vi "Main_RT_V2.vi"() -> ()   [LabVIEW 2018]
uses:
  enum_Main_RT_V2.ctl
  <vilib>/Platform/TimedLoop/XDataNode/timing_clust.ctl
  <vilib>/Platform/TimedLoop/XDataNode/nitl_modes.ctl
  <vilib>/Platform/TimedLoop/XDataNode/wakeup.ctl
  enum_bras.ctl
  <vilib>/myRIO/Instrument Drivers/Onboard IO/DIO/typedefs/DIO Reference.ctl
  <vilib>/myRIO/Common/Instrument Driver Framework/Utilities/typedefs/myRIO Generic Hardware Reference.ctl
  <vilib>/myRIO/Common/Instrument Driver Framework/Utilities/typedefs/Hardware Version Enum.ctl
  <vilib>/myRIO/Common/Instrument Driver Framework/Utilities/typedefs/myRIO v1.0 Reference.ctl
  <vilib>/myRIO/Common/Instrument Driver Framework/Utilities/typedefs/Generic FPGA Reference.ctl
  <vilib>/myRIO/Common/Instrument Driver Framework/myRIO v1.0/DIO/typedefs/DIO Channels List.ctl
  <vilib>/myRIO/Common/Instrument Driver Framework/myRIO v1.0/DIO/typedefs/DIO Channels Enum.ctl
  <vilib>/userdefined/High Color/nirio_resource_hc.ctl
  enum_RT_Virage.ctl
  enum_RT_Seaux.ctl
  enum_RT_recule.ctl
  enum_RT_trieur_Balles.ctl
  enum_RT_lanceur.ctl
  <vilib>/myRIO/Common/Instrument Driver Framework/Utilities/vis/Is FPGA Ref Available.vi
  <vilib>/myRIO/Common/Instrument Driver Framework/myRIO v1.0/DIO/vis/myRIO v1.1 Open DIO.vi
  <vilib>/myRIO/Instrument Drivers/Onboard IO/DIO/vis/Read.vi
  <vilib>/myRIO/Instrument Drivers/Onboard IO/DIO/vis/Write.vi
  <vilib>/myRIO/Common/Instrument Driver Framework/Utilities/vis/Validate Channels.vi
  <vilib>/myRIO/Common/Instrument Driver Framework/myRIO v1.0/DIO/vis/myRIO v1.0 Reserve DIO.vi
  <vilib>/myRIO/Common/Instrument Driver Framework/myRIO v1.0/Resource Manager/vis/myRIO v1.0 Reserve Channel List.vi
  <vilib>/myRIO/Common/Instrument Driver Framework/myRIO v1.0/DIO/vis/myRIO v1.0 Build MUX Configuration DIO.vi
  <vilib>/myRIO/Common/Instrument Driver Framework/myRIO v1.0/Resource Manager/vis/myRIO v1.0 Reserve Channel.vi
  <vilib>/myRIO/Common/Instrument Driver Framework/myRIO v1.0/Resource Manager/vis/myRIO v1.0 Unreserve Channel.vi
  <vilib>/myRIO/Common/Instrument Driver Framework/myRIO v1.0/Resource Manager/vis/myRIO v1.0 Create Configuration List.vi
  <vilib>/myRIO/Common/Instrument Driver Framework/myRIO v1.0/Resource Manager/vis/myRIO v1.0 Build Mutex Name.vi
  <vilib>/Utility/VariantDataType/GetNumericInfo.vi
  <vilib>/Utility/error.llb/Error Cluster From Error Code.vi
  <vilib>/myRIO/Common/Instrument Driver Framework/myRIO v1.0/myRIO v1.1 Open.vi
  <vilib>/myRIO/Common/Instrument Driver Framework/Utilities/vis/IO Manager.vi
  <vilib>/myRIO/Common/Instrument Driver Framework/Utilities/vis/Configuration Manager.vi
  <vilib>/myRIO/Common/Instrument Driver Framework/myRIO v1.0/Resource Manager/vis/myRIO v1.0 Configure IO.vi
  <vilib>/myRIO/Common/Instrument Driver Framework/myRIO v1.0/myRIO v1.0 Close.vi
  <vilib>/myRIO/Common/Instrument Driver Framework/myRIO v1.0/DIO/vis/myRIO v1.0 Read DIO.vi
  <vilib>/myRIO/Common/Instrument Driver Framework/myRIO v1.0/DIO/vis/myRIO v1.0 Write DIO.vi
  <vilib>/Platform/TimedLoop/XDataNode/XDataNode.xnode
  <vilib>/myRIO/Express VI/Onboard Devices/Button/Button Express VI.xnode
  <vilib>/myRIO/Instrument Drivers/Onboard IO/DIO/vis/myRIO DIO Open.xnode
  <vilib>/myRIO/Express VI/Onboard Devices/LED/LED Express VI.xnode
  <vilib>/Platform/TimedLoop/XDataNode/XDNodeRunTimeDep.lvlib
  <vilib>/myRIO/Instrument Drivers/Onboard IO/DIO/DIO.lvlib
panel:
  in  "lancer le robot":bool
  in  "stop":bool
  out "Sceaux":bool
  out "Lanceur de balles":bool
  out "Virage 4":bool
  out "Virage 3":bool
  out "Clapets 2":bool
  out "Trieur de Balles":bool
  out "Reculer":bool
  out "Virage 2":bool
  out "Virage 1":bool
  out "Clapets 1":bool
  out "Detection suiveur de ligne":bool[](array[boolean])
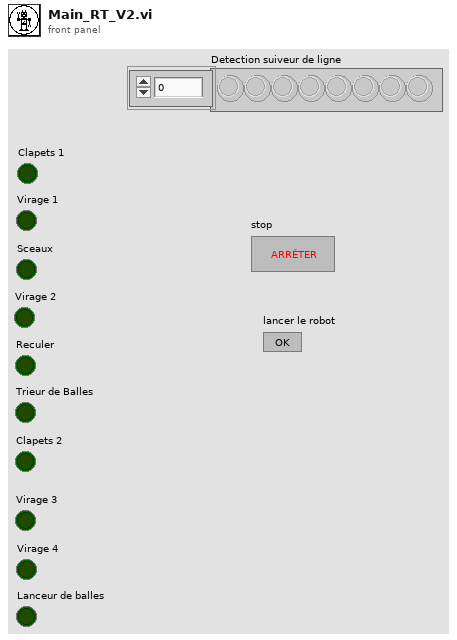
[diagram p1: front panel]
types:
  T1 = typedef "enum_Main_RT_V2.ctl" = enum16{"Initialisation", "Clapet 1", "Virage 1", "Seaux", "Virage 2", "Reculer", "Trieur Balles", "Avancer", "Clapet 2", "Virage 3", "Avancer 2", "Virage 4", "Lancer de Balles", "Arret du robot"}
  T2 = typedef "XDNodeRunTimeDep.lvlib/timing_clust.ctl" = cluster{"Expected End [f-1]":u64, "Actual End [f-1]":u64, "Finished Late? [f-1]":bool, "Expected End [i-1]":u64, "Actual End [i-1]":u64, "Finished Late? [i-1]":bool, "Expected Start [i]":u64, "Actual Start [i]":u64, "Expected Start [f]":u64, "Actual Start [f]":u64, "Source Name":string, "Structure Name":string, "Period":i64, "Deadline":i64, "Offset":i64, "Start":i64, "Priority":i32, "Timeout":i32, "Mode":T3, "Wakeup Reason":T4, "Error":errorcluster, "Source Type":string, "Secondary Source Type":string, "Global End Time":u64, "Global Start Time":u64, "Frame Duration":u64, "Iteration Duration":u64, "Assigned CPU":i32, "I/O Scan Engine Mode":u32}
  T3 = typedef "XDNodeRunTimeDep.lvlib/nitl_modes.ctl" = enum32{"No Change", "Process missed periods, maintain original phase", "Discard missed periods, maintain original phase", "Process missed periods, ignore original phase", "Discard missed periods, ignore original phase"}
  T4 = typedef "XDNodeRunTimeDep.lvlib/wakeup.ctl" = enum32{"Normal", "Aborted", "Asynchronous wakeup", "Timing source error", "Timed loop error", "Timeout"}
  T5 = typedef "enum_bras.ctl" = enum16{"Depart Bras", "Clapet Bras", "Inactif Bras", "Seaux Bras"}
  T6 = typedef "DIO.lvlib/DIO Reference.ctl" = cluster{"myRIO Reference":T7, "DIO Channels List":T11}
  T7 = typedef "myRIO Generic Hardware Reference.ctl" = cluster{"myRIO Model":T8, "myRIO Hardware Reference":T9}
  T8 = typedef "Hardware Version Enum.ctl" = enum16{"Unknown", "myRIO-1900", "myRIO-1950", "roboRIO", "NI ELVIS RIO CM", "ELVIS III"}
  T9 = typedef "myRIO v1.0 Reference.ctl" = cluster{"Generic FPGA Reference":T10, "Allow multiple opens":bool}
  T10 = typedef "Generic FPGA Reference.ctl" = refnum<k20>
  T11 = typedef "DIO Channels List.ctl" = T12[]
  T12 = typedef "DIO Channels Enum.ctl" = enum16{"Not Connected", "C/DIO0", "C/DIO1", "C/DIO2", "C/DIO3", "C/DIO4", "C/DIO5", "C/DIO6", "C/DIO7", "A/DIO0", "A/DIO1", "A/DIO2", "A/DIO3", "A/DIO4", "A/DIO5", "A/DIO6", "A/DIO7", "A/DIO8", "A/DIO9", "A/DIO10", "A/DIO11", "A/DIO12", "A/DIO13", "A/DIO14", "A/DIO15", "A/DIO16", "A/DIO17", "A/DIO18", "A/DIO19", "B/DIO0", "B/DIO1", "B/DIO2", "B/DIO3", "B/DIO4", "B/DIO5", "B/DIO6", "B/DIO7", "B/DIO8", "B/DIO9", "B/DIO10", "B/DIO11", "B/DIO12", "B/DIO13", "B/DIO14", "B/DIO15", "B/DIO16", "B/DIO17", "B/DIO18", "B/DIO19", "LED0", "LED1", "LED2", "LED3", "Button0", "DIO/DIO0", "DIO/DIO1", "DIO/DIO2", "DIO/DIO3", "DIO/DIO4", "DIO/DIO5", "DIO/DIO6", "DIO/DIO7", "DIO/DIO8", "DIO/DIO9", "SPI/CS0", "SPI/CS1", "SPI/CS2", "SPI/CS3", "LED RADIO (Green)", "LED RADIO (Red)", "LED COMM (Green)", "LED COMM (Red)", "LED MODE (Green)", "LED MODE (Red)"}
  T13 = typedef "nirio_resource_hc.ctl" = tag
  T14 = typedef "enum_RT_Virage.ctl" = enum16{"Avancer", "STOP", "Lacher Ligne", "Tourner"}
  T15 = typedef "enum_RT_Seaux.ctl" = enum16{"Avancé 1", "Ready to Start", "Stop moteur", "Bras Inactif 1", "Frappe sceau", "Bras Inactif 2", "Avancé 2"}
  T16 = typedef "enum_RT_recule.ctl" = enum16{"Avancer", "Reculer", "STOP"}
  T17 = typedef "enum_RT_trieur_Balles.ctl" = enum16{"Initialisation", "Couleur", "Rotation1", "Rotation2", "Ouverture", "Fermeture"}
  T18 = typedef "enum_RT_lanceur.ctl" = enum16{"eloignement", "arret_robot", "moteur_lanceur", "distributeur", "arret_distributeur_lanceur"}
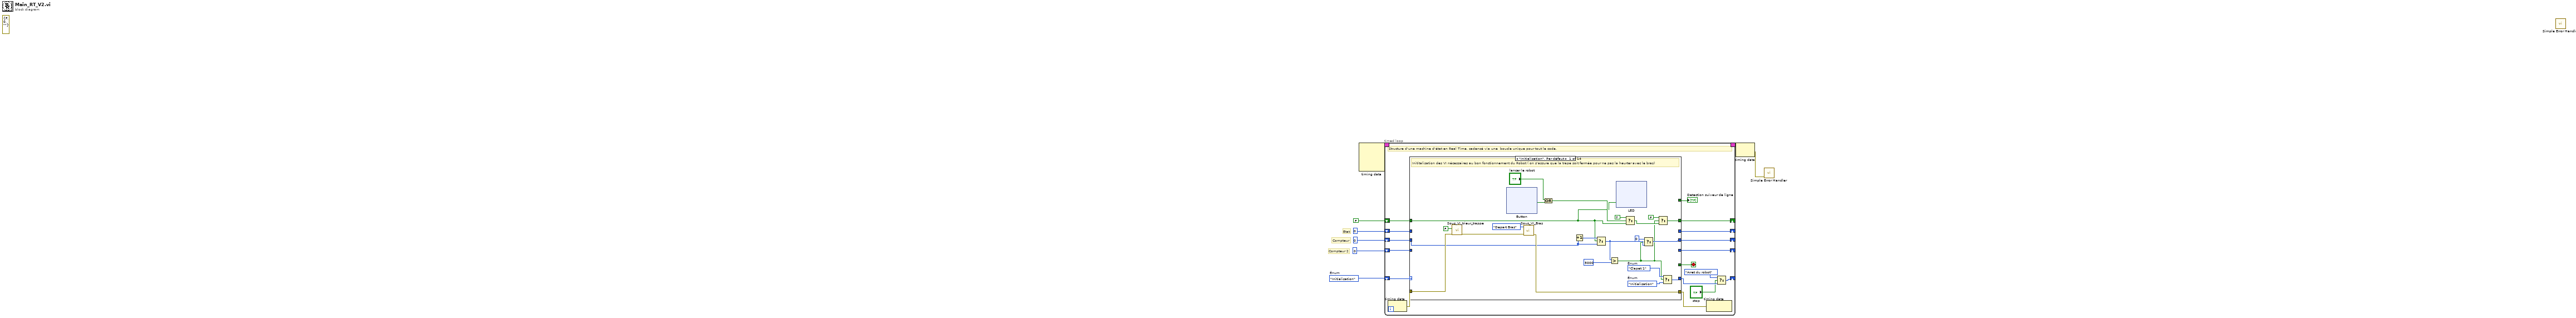
[diagram p0: block diagram]
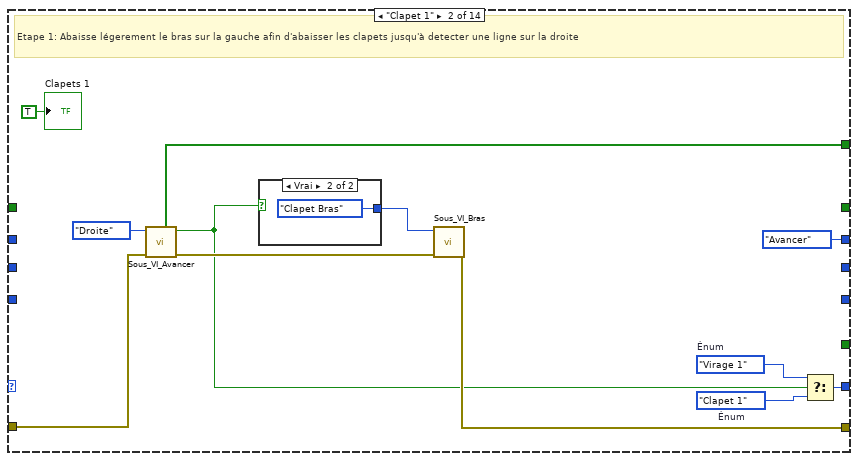
[diagram p2: hidden frame]
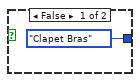
[diagram p3: hidden frame]
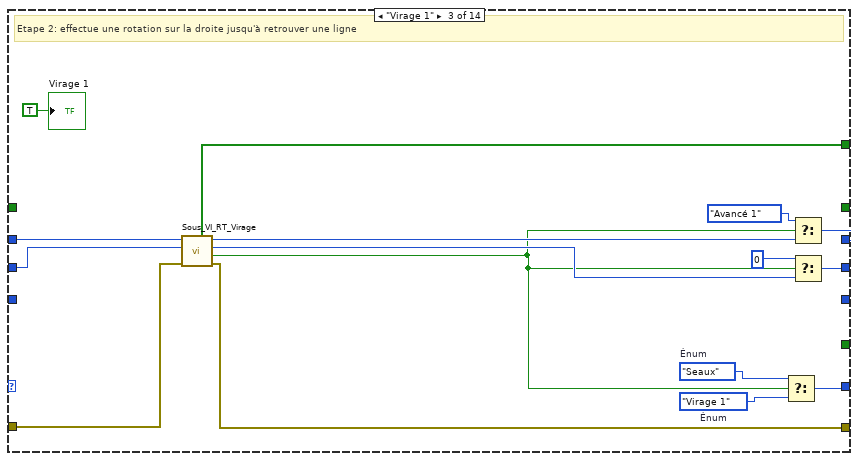
[diagram p4: hidden frame]
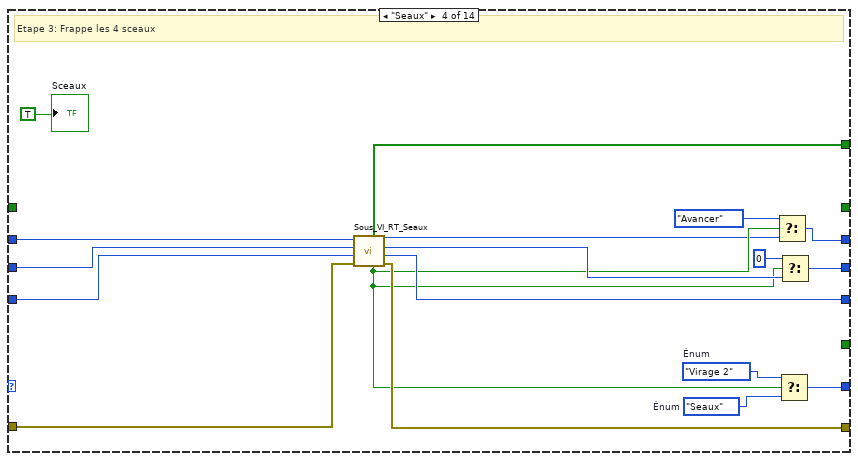
[diagram p5: hidden frame]
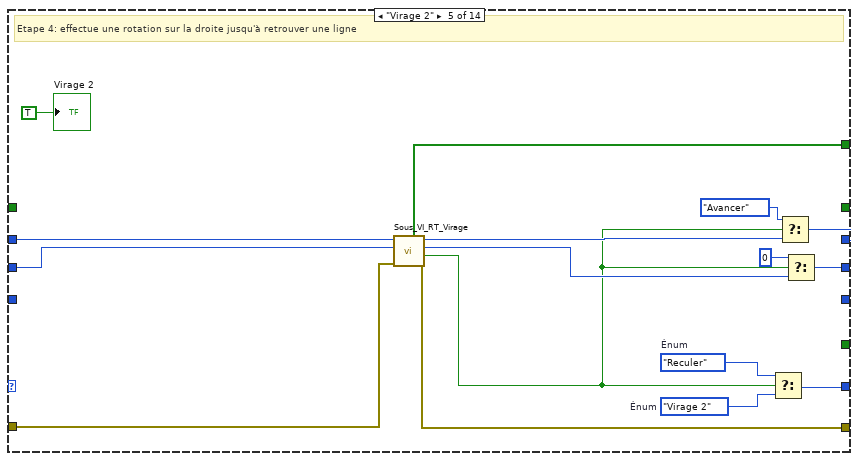
[diagram p6: hidden frame]
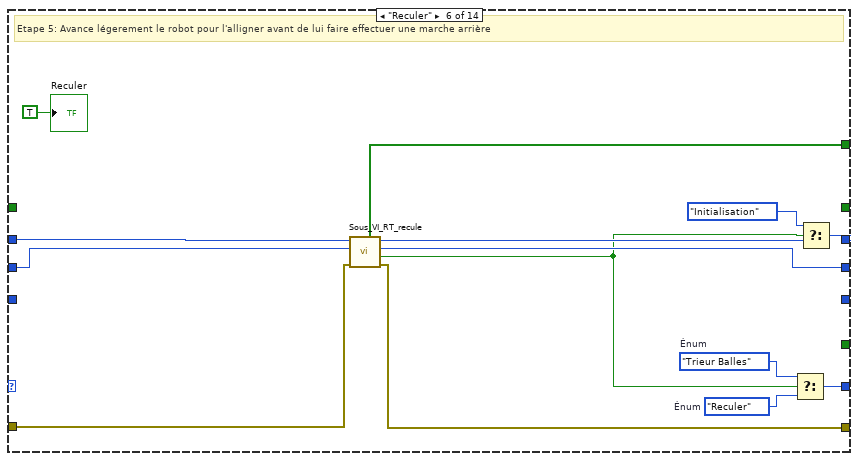
[diagram p7: hidden frame]
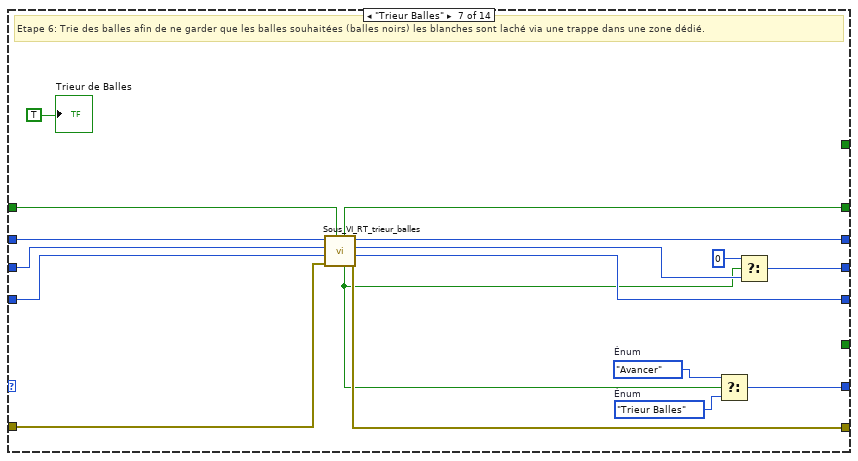
[diagram p8: hidden frame]
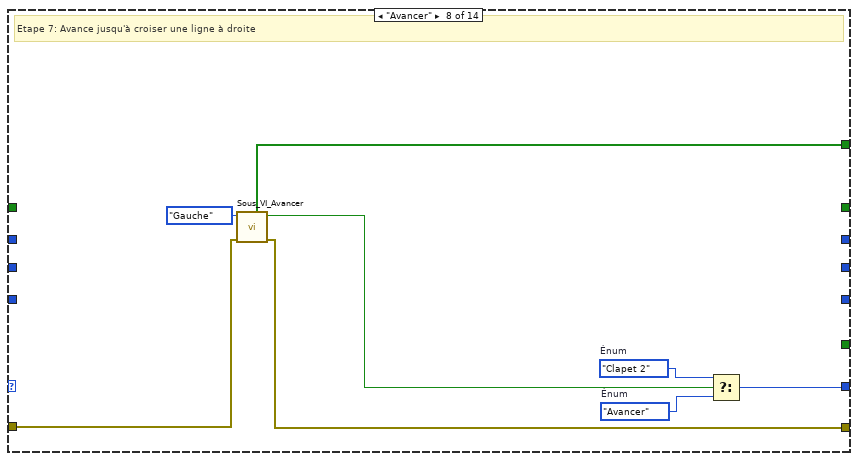
[diagram p9: hidden frame]
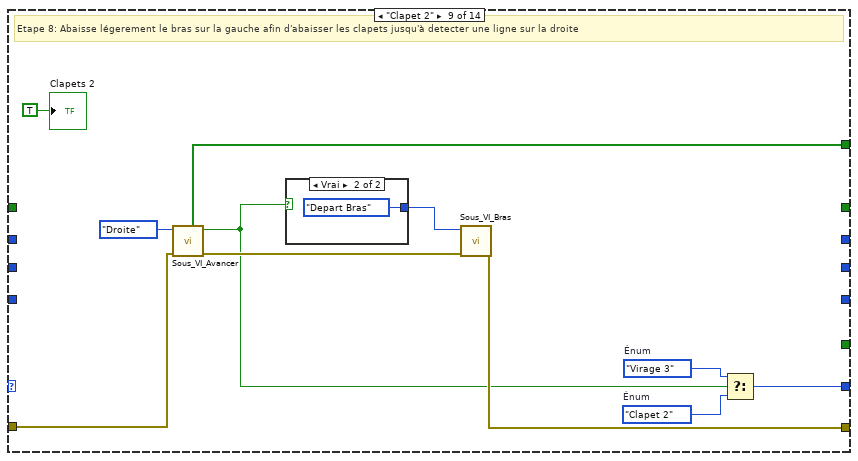
[diagram p10: hidden frame]
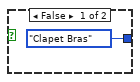
[diagram p11: hidden frame]
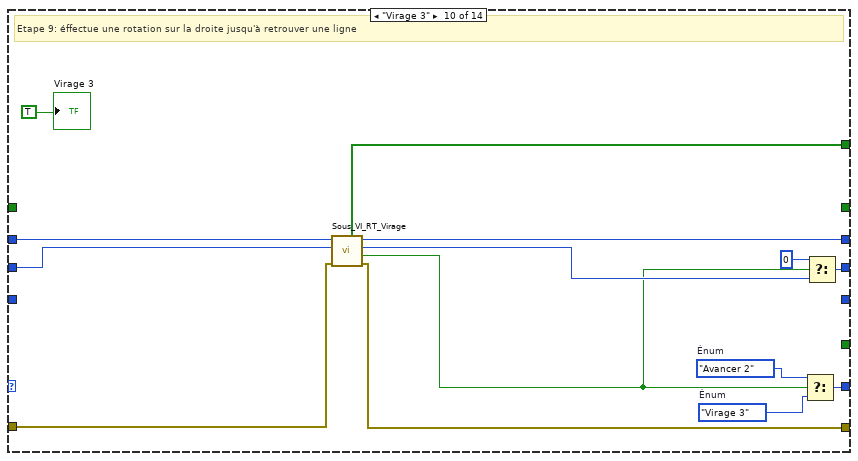
[diagram p12: hidden frame]
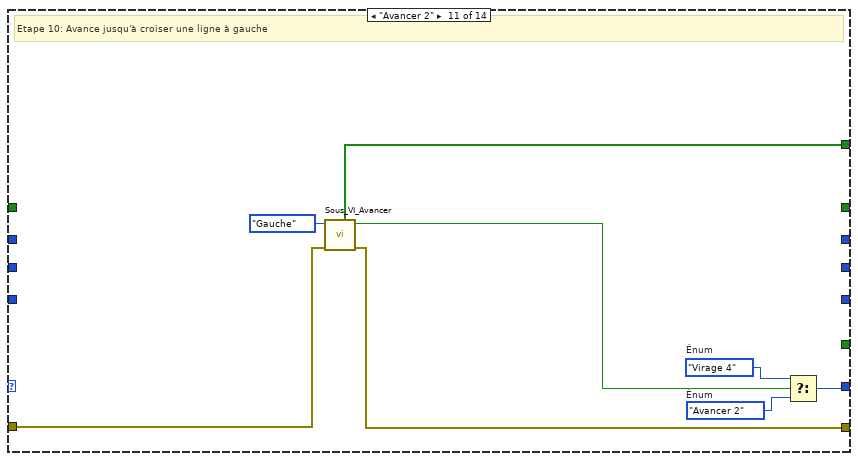
[diagram p13: hidden frame]
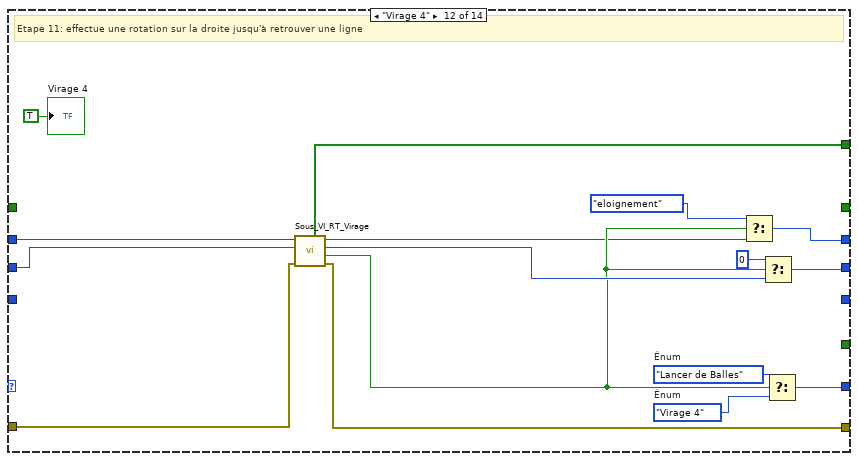
[diagram p14: hidden frame]
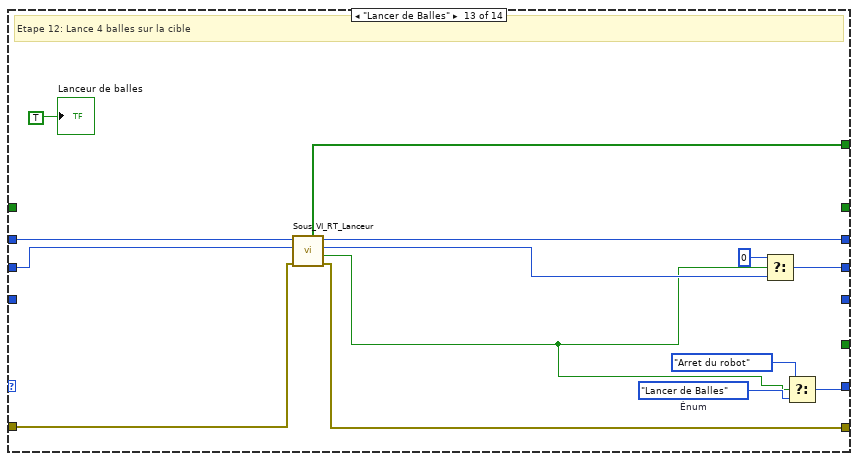
[diagram p15: hidden frame]
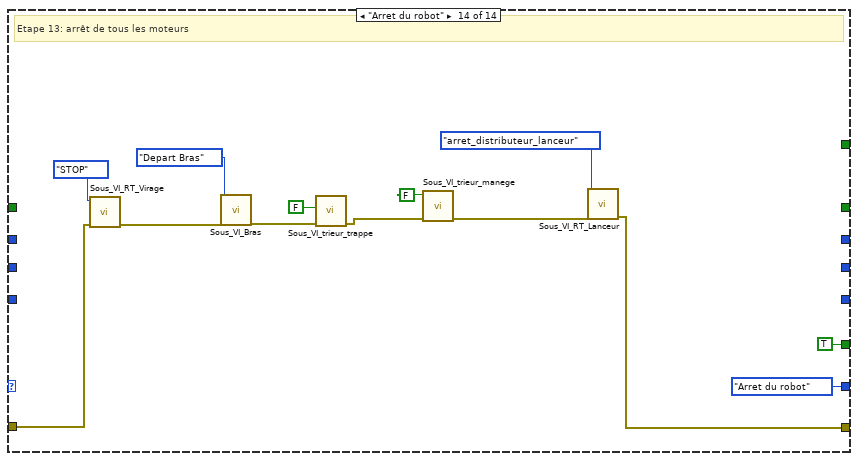
[diagram p16: hidden frame]
diagram:
  w1 = enum_Main_RT_V2."Initialisation"  # Énum
  (unwired) errorcluster {"status"=FALSE, "code"=0, "source"=""} ("error in (no error)")
  # "Compteur 2"
  # "Compteur"
  # "Etat"
  n1 = node-c288() -> (w8:T2)  [unwired: 4 in]
  n2 = timed-loop "Boucle cadencée" {
    timing: w8 -> [_]
    timing-out: [_] -> w7
    shift-right: [w22] -> _
    shift-left: u16 0 ("Etat OUT") -> [w20]
    shift-right: [w21] -> _
    shift-left: 0 -> [w19]
    shift-right: [w17] -> _
    shift-left: 0 -> [w18]
    shift-right: [w15] -> _
    shift-left: FALSE -> [w16]
    shift-right: [w12] -> _
    shift-left: w1 -> [w25]
    stop <- w14 stop-if-true
    # "Structure d'une machine d'état en Real Time, cadencé via une  boucle unique pour tout le code."
    n3 = node-c288() -> (w24:errorcluster)  [unwired: 1 in]
    n4 = case "Structure Condition" shown="\"Initialisation\", Par défaut" w25 {
      tunnel: w24 -> [w45 w127 w148 w166 w182 w193 w206 w220 w229 w245 w255 w270 w273 w299]
      tunnel: [w44 w126 w147 w165 w181 w192 w205 w219 w228 w244 w254 w269 w283 w289] -> w23
      tunnel: [_ enum_RT_Virage."Avancer" ("Etat IN") w139 w152 w170 w186 w212 _ _ w246 _ w260 w285 _] -> w22
      tunnel: [w34 _ w145 w161 w177 w194 w203 _ _ w242 _ w267 w281 _] -> w21
      tunnel: w20 -> [_ _ w141 w157 w180 w196 w213 _ _ w248 _ w272 w286 _]
      tunnel: w19 -> [w36 _ w146 w164 w179 w195 w211 _ _ w247 _ w271 w284 _]
      tunnel: w18 -> [_ _ _ w163 _ _ w210 _ _ _ _ _ _ _]
      tunnel: [_ _ _ w162 _ _ w209 _ _ _ _ _ _ _] -> w17
      tunnel: w16 -> [w26 _ _ _ _ _ w208 _ _ _ _ _ _ _]
      tunnel: [w30 _ _ _ _ _ w207 _ _ _ _ _ _ _] -> w15
      tunnel: [_ _ _ _ _ _ _ _ _ _ _ _ _ TRUE ("vi_fini")] -> w14
      tunnel: [w43 w122 w136 w156 w173 w190 w199 w218 w227 w238 w253 w264 w277 enum_Main_RT_V2."Arret du robot" ("Énum")] -> w11
      tunnel: [_ w124 w142 w158 w175 w191 _ w217 w225 w239 w251 w265 w279 _] -> w13
      frame "Initialisation", Default {
        w41 = enum_Main_RT_V2."Clapet 1"  # Énum
        w42 = enum_Main_RT_V2."Initialisation"  # Énum
        # "Inititalisation des VI nécessaires au bon fonctionnement du Robot ( on s'assure que la trape soit fermée pour ne pas la heurter avec le bras)"
        n5 = call "Sous_VI_trieur_trappe.vi"("error in (no error)"=w45, "Ouvrir"=FALSE) -> ("error out"=w46:errorcluster)  [unwired: 9 in]
        n6 = xnode "Button"() -> ("Value"=w40:bool)  [unwired: 1 in, 1 out]
        n7 = call "Sous_VI_Bras.vi"("error in (no error)"=w46, "Enum bras"=enum_bras."Depart Bras") -> ("error out"=w44:errorcluster)  [unwired: 9 in]
        n8 = Or(x="lancer le robot", y=w40) -> (x .or. y?=w37:bool)
        n9 = Increment(x=w36) -> (x+1=w35:i32)
        n10 = Select(t=w35, s=w26, f=w36) -> (s? t:f=w32:i32)
        n11 = Greater?(x=w32, y=5000 ("delay")) -> (0:w28:bool)
        n12 = xnode "LED"("LED0"=w26) -> ()  [unwired: 1 in, 1 out]
        n13 = Select(t=TRUE ("cas vrai"), s=w37, f=w26) -> (s? t:f=w29:bool)
        n14 = Select(t=0 ("cas vrai"), s=w28, f=w32) -> (s? t:f=w34:i32)
        n15 = Select(t=FALSE ("cas vrai"), s=w28, f=w29) -> (s? t:f=w30:bool)
        n16 = Select(t=w41, s=w28, f=w42) -> (s? t:f=w43:T1)
      }
      frame "Clapet 1" {
        w120 = enum_Main_RT_V2."Clapet 1"  # Énum
        w119 = enum_Main_RT_V2."Virage 1"  # Énum
        # "Etape 1: Abaisse légerement le bras sur la gauche afin d'abaisser les clapets jusqu'à detecter une ligne sur la droite"
        n17 = call "Sous_VI_Avancer.vi"("error in (no error)"=w127, "Énum"=enum16{"Droite", "Gauche"}."Droite") -> ("error out"=w128:errorcluster, "Info de fin de Parcours"=w125:bool, "Détection ligne"=w124:bool[])  [unwired: 7 in]
        n18 = case shown="Vrai" w125 {
          tunnel: [enum_bras."Clapet Bras" ("Enum bras") enum_bras."Clapet Bras" ("Enum bras")] -> w129
          frame False {
          }
          frame True {
          }
        }
        n19 = call "Sous_VI_Bras.vi"("error in (no error)"=w128, "Enum bras"=w129) -> ("error out"=w126:errorcluster)  [unwired: 9 in]
        n20 = Select(t=w119, s=w125, f=w120) -> (s? t:f=w122:T1)
        "Clapets 1" <- TRUE
      }
      frame "Virage 1" {
        w134 = enum_Main_RT_V2."Virage 1"  # Énum
        w133 = enum_Main_RT_V2."Seaux"  # Énum
        # "Etape 2: effectue une rotation sur la droite jusqu'à retrouver une ligne"
        n21 = call "Sous_VI_RT_Virage.vi"("Erreur in"=w148, "Compteur IN"=w146, "Etat IN"=w141) -> ("Erreur out"=w147:errorcluster, "Information de fin de process"=w138:bool, "Compteur OUT"=w143:i32, "Etat OUT"=w140:T14, "Detection suiveur de ligne"=w142:bool[])  [unwired: 4 in]
        n22 = Select(t=w133, s=w138, f=w134) -> (s? t:f=w136:T1)
        n23 = Select(t=enum_RT_Seaux."Avancé 1" ("Etat IN"), s=w138, f=w140) -> (s? t:f=w139:u16)
        n24 = Select(t=0, s=w138, f=w143) -> (s? t:f=w145:i32)
        "Virage 1" <- TRUE
      }
      frame "Seaux" {
        w153 = enum_Main_RT_V2."Seaux"  # Énum
        w154 = enum_Main_RT_V2."Virage 2"  # Énum
        # "Etape 3: Frappe les 4 sceaux"
        n25 = call "Sous_VI_RT_Seaux.vi"("Erreur IN"=w166, "Nombre Sceau IN"=w163, "Compteur IN"=w164, "Etat IN"=w157) -> ("Erreur OUT"=w165:errorcluster, "Nombre Sceau OUT"=w162:i32, "Compteur OUT"=w159:i32, "Etat OUT"=w149:T15, "Indicateur de fin de process"=w151:bool, "Détection ligne"=w158:bool[])  [unwired: 2 in]
        n26 = Select(t=enum_RT_Virage."Avancer" ("Etat IN"), s=w151, f=w149) -> (s? t:f=w152:u16)
        n27 = Select(t=w154, s=w151, f=w153) -> (s? t:f=w156:T1)
        n28 = Select(t=0, s=w151, f=w159) -> (s? t:f=w161:i32)
        "Sceaux" <- TRUE
      }
      frame "Virage 2" {
        w171 = enum_Main_RT_V2."Reculer"  # Énum
        w172 = enum_Main_RT_V2."Virage 2"  # Énum
        # "Etape 4: effectue une rotation sur la droite jusqu'à retrouver une ligne"
        n29 = call "Sous_VI_RT_Virage.vi"("Erreur in"=w182, "Compteur IN"=w179, "Etat IN"=w180) -> ("Erreur out"=w181:errorcluster, "Information de fin de process"=w168:bool, "Compteur OUT"=w176:i32, "Etat OUT"=w169:T14, "Detection suiveur de ligne"=w175:bool[])  [unwired: 4 in]
        n30 = Select(t=w171, s=w168, f=w172) -> (s? t:f=w173:T1)
        n31 = Select(t=enum_RT_recule."Avancer", s=w168, f=w169) -> (s? t:f=w170:u16)
        n32 = Select(t=0, s=w168, f=w176) -> (s? t:f=w177:i32)
        "Virage 2" <- TRUE
      }
      frame "Reculer" {
        w188 = enum_Main_RT_V2."Reculer"  # Énum
        w187 = enum_Main_RT_V2."Trieur Balles"  # Énum
        # "Etape 5: Avance légerement le robot pour l'alligner avant de lui faire effectuer une marche arrière"
        n33 = call "Sous_VI_RT_recule.vi"("Erreur IN"=w193, "Compteur IN"=w195, "Etat IN"=w196) -> ("Erreur OUT"=w192:errorcluster, "Indicateur fin de process"=w183:bool, "Compteur OUT"=w194:i32, "Etat OUT"=w185:T16, "Detection suiveur de ligne"=w191:bool[])  [unwired: 4 in]
        n34 = Select(t=w187, s=w183, f=w188) -> (s? t:f=w190:T1)
        n35 = Select(t=enum_RT_trieur_Balles."Initialisation", s=w183, f=w185) -> (s? t:f=w186:u16)
        "Reculer" <- TRUE
      }
      frame "Trieur Balles" {
        w197 = enum_Main_RT_V2."Avancer"  # Énum
        w198 = enum_Main_RT_V2."Trieur Balles"  # Énum
        # "Etape 6: Trie des balles afin de ne garder que les balles souhaitées (balles noirs) les blanches sont laché via une trappe dans une zone dédié."
        n36 = call "Sous_VI_RT_trieur_balles.vi"("Détection couleur IN"=w208, "error in (no error)"=w206, "Nombre Balle IN"=w210, "Comteur IN"=w211, "Etat IN"=w213) -> ("error out"=w205:errorcluster, "Nombre Balle OUT"=w209:i32, "Comteur OUT"=w202:i32, "Etat OUT"=w212:T17, "Indicateur de fin de process"=w201:bool, "Détection couleur OUT"=w207:bool)  [unwired: 1 in]
        n37 = Select(t=w197, s=w201, f=w198) -> (s? t:f=w199:T1)
        n38 = Select(t=0, s=w201, f=w202) -> (s? t:f=w203:i32)
        "Trieur de Balles" <- TRUE
      }
      frame "Avancer" {
        w215 = enum_Main_RT_V2."Clapet 2"  # Énum
        w216 = enum_Main_RT_V2."Avancer"  # Énum
        # "Etape 7: Avance jusqu'à croiser une ligne à droite"
        n39 = call "Sous_VI_Avancer.vi"("error in (no error)"=w220, "Énum"=enum16{"Droite", "Gauche"}."Gauche") -> ("error out"=w219:errorcluster, "Info de fin de Parcours"=w214:bool, "Détection ligne"=w217:bool[])  [unwired: 7 in]
        n40 = Select(t=w215, s=w214, f=w216) -> (s? t:f=w218:T1)
      }
      frame "Clapet 2" {
        w222 = enum_Main_RT_V2."Virage 3"  # Énum
        w223 = enum_Main_RT_V2."Clapet 2"  # Énum
        # "Etape 8: Abaisse légerement le bras sur la gauche afin d'abaisser les clapets jusqu'à detecter une ligne sur la droite"
        n41 = call "Sous_VI_Avancer.vi"("error in (no error)"=w229, "Énum"=enum16{"Droite", "Gauche"}."Droite") -> ("error out"=w230:errorcluster, "Info de fin de Parcours"=w226:bool, "Détection ligne"=w225:bool[])  [unwired: 7 in]
        n42 = case shown="Vrai" w226 {
          tunnel: [enum_bras."Clapet Bras" ("Enum bras") enum_bras."Depart Bras" ("Enum bras")] -> w231
          frame False {
          }
          frame True {
          }
        }
        n43 = call "Sous_VI_Bras.vi"("error in (no error)"=w230, "Enum bras"=w231) -> ("error out"=w228:errorcluster)  [unwired: 9 in]
        n44 = Select(t=w222, s=w226, f=w223) -> (s? t:f=w227:T1)
        "Clapets 2" <- TRUE
      }
      frame "Virage 3" {
        w235 = enum_Main_RT_V2."Avancer 2"  # Énum
        w236 = enum_Main_RT_V2."Virage 3"  # Énum
        # "Etape 9: éffectue une rotation sur la droite jusqu'à retrouver une ligne"
        n45 = call "Sous_VI_RT_Virage.vi"("Erreur in"=w245, "Compteur IN"=w247, "Etat IN"=w248) -> ("Erreur out"=w244:errorcluster, "Information de fin de process"=w240:bool, "Compteur OUT"=w241:i32, "Etat OUT"=w246:T14, "Detection suiveur de ligne"=w239:bool[])  [unwired: 4 in]
        n46 = Select(t=w235, s=w240, f=w236) -> (s? t:f=w238:T1)
        n47 = Select(t=0, s=w240, f=w241) -> (s? t:f=w242:i32)
        "Virage 3" <- TRUE
      }
      frame "Avancer 2" {
        w249 = enum_Main_RT_V2."Virage 4"  # Énum
        w250 = enum_Main_RT_V2."Avancer 2"  # Énum
        # "Etape 10: Avance jusqu'à croiser une ligne à gauche"
        n48 = call "Sous_VI_Avancer.vi"("error in (no error)"=w255, "Énum"=enum16{"Droite", "Gauche"}."Gauche") -> ("error out"=w254:errorcluster, "Info de fin de Parcours"=w252:bool, "Détection ligne"=w251:bool[])  [unwired: 7 in]
        n49 = Select(t=w249, s=w252, f=w250) -> (s? t:f=w253:T1)
      }
      frame "Virage 4" {
        w262 = enum_Main_RT_V2."Lancer de Balles"  # Énum
        w261 = enum_Main_RT_V2."Virage 4"  # Énum
        # "Etape 11: effectue une rotation sur la droite jusqu'à retrouver une ligne"
        n50 = call "Sous_VI_RT_Virage.vi"("Erreur in"=w270, "Compteur IN"=w271, "Etat IN"=w272) -> ("Erreur out"=w269:errorcluster, "Information de fin de process"=w259:bool, "Compteur OUT"=w266:i32, "Etat OUT"=w257:T14, "Detection suiveur de ligne"=w265:bool[])  [unwired: 4 in]
        n51 = Select(t=enum_RT_lanceur."eloignement", s=w259, f=w257) -> (s? t:f=w260:u16)
        n52 = Select(t=0, s=w259, f=w266) -> (s? t:f=w267:i32)
        n53 = Select(t=w262, s=w259, f=w261) -> (s? t:f=w264:T1)
        "Virage 4" <- TRUE ("Virage 4")
      }
      frame "Lancer de Balles" {
        w276 = enum_Main_RT_V2."Lancer de Balles"  # Énum
        # "Etape 12: Lance 4 balles sur la cible"
        n54 = call "Sous_VI_RT_Lanceur.vi"("Erreur_in"=w273, "cpt_in"=w284, "enum_in"=w286) -> ("Erreur_out"=w283:errorcluster, "vi_fini"=w274:bool, "cpt_out"=w280:i32, "enum_out"=w285:T18, "Détection de ligne"=w279:bool[])  [unwired: 4 in]
        n55 = Select(t=0, s=w274, f=w280) -> (s? t:f=w281:i32)
        n56 = Select(t=enum_Main_RT_V2."Arret du robot" ("cas vrai"), s=w274, f=w276) -> (s? t:f=w277:T1)
        "Lanceur de balles" <- TRUE
      }
      frame "Arret du robot" {
        # "Etape 13: arrêt de tous les moteurs"
        n57 = call "Sous_VI_RT_Virage.vi"("Erreur in"=w299, "Etat IN"=enum_RT_Virage."STOP") -> ("Erreur out"=w298:errorcluster)  [unwired: 5 in, 4 out]
        n58 = call "Sous_VI_Bras.vi"("error in (no error)"=w298, "Enum bras"=enum_bras."Depart Bras") -> ("error out"=w294:errorcluster)  [unwired: 9 in]
        n59 = call "Sous_VI_trieur_trappe.vi"("error in (no error)"=w294, "Ouvrir"=FALSE) -> ("error out"=w292:errorcluster)  [unwired: 9 in]
        n60 = call "Sous_VI_trieur_manege.vi"("error in (no error)"=w292, "ON/OFF"=FALSE) -> ("error out"=w291:errorcluster)  [unwired: 9 in]
        n61 = call "Sous_VI_RT_Lanceur.vi"("Erreur_in"=w291, "enum_in"=enum_RT_lanceur."arret_distributeur_lanceur") -> ("Erreur_out"=w289:errorcluster)  [unwired: 5 in, 4 out]
      }
    }
    "Detection suiveur de ligne" <- w13
    n62 = node-c288(w23) -> ()  [unwired: 1 out]
    n63 = Select(t=enum_Main_RT_V2."Arret du robot" ("cas vrai"), s="stop", f=w11) -> (s? t:f=w12:T1)
  }
  n64 = node-c288(w7) -> (w3:errorcluster)
  n65 = call <vilib>:"Simple Error Handler.vi"("error in (no error)"=w3) -> ()  [unwired: 4 in, 5 out]
  n66 = call <vilib>:"Simple Error Handler.vi"() -> ()  [unwired: 5 in, 5 out]
